vi "Set Scale.vi"(9 "Scale Visible":bool[](array[boolean]), 10 "X坐标轴":T1, 11 "Data Viewer in":refnum<class "Data Viewer.lvclass">) -> (3 "Data Viewer Out":refnum<class "Data Viewer.lvclass">)   [LabVIEW 2020, in "Data Viewer.lvlib" / "Data Viewer.lvclass"]
uses:
  Data Viewer.lvclass
  Data Viewer.lvclass/Data Viewer.ctl
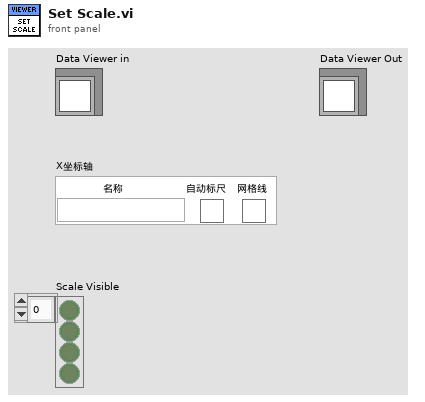
[diagram p1: front panel]
types:
  T1 = cluster{"名称":string, "Auto Scale":bool, "Gird Line":bool}
  T2 = typedef "Data Viewer.lvlib/Data Viewer.lvclass/Scale Setting--cluster.ctl" = cluster{"Name":string, "Unit":string, "Color":u32, "Auto Scale":bool, "Scale Min":dbl, "Scale Max":dbl, "Scale Interval":dbl, "Show Gird":bool, "Log":bool}
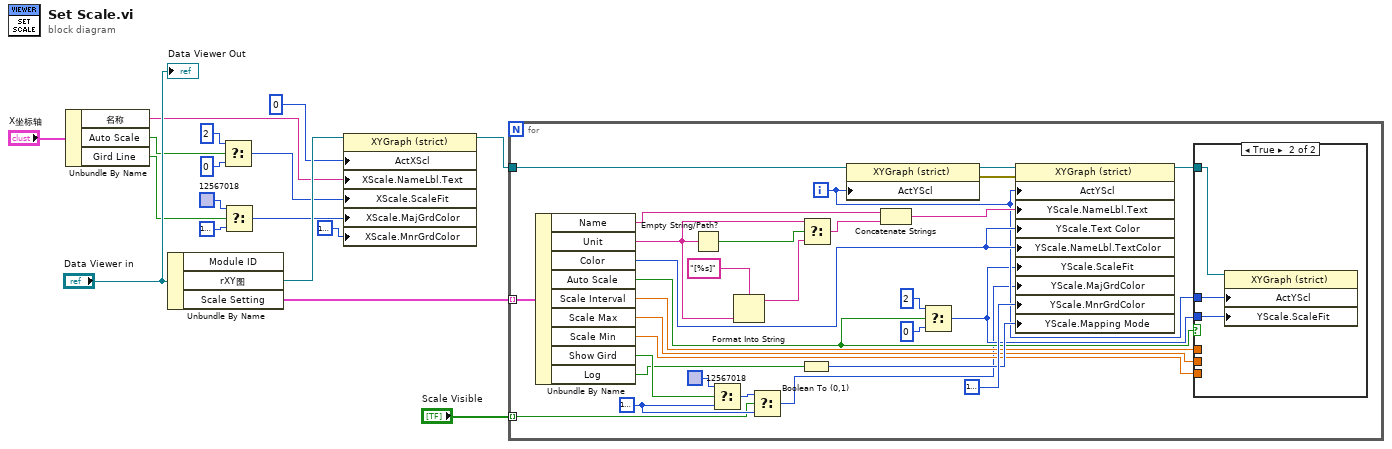
[diagram p0: block diagram]
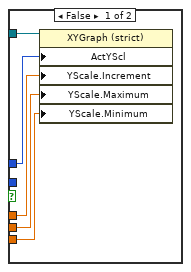
[diagram p2: hidden frame]
diagram:
  n1 = Unbundle By Name("X坐标轴") -> ("名称"=w12:string, "Auto Scale"=w11:bool, "Gird Line"=w6:bool)
  n2 = Unbundle By Name("Data Viewer in") -> ("rXY图"=w15:refnum<vi>, "Scale Setting"=w17:T2[])  [unwired: 1 out]
  n3 = Select(t=u8 2, s=w11, f=u8 0 ("Y Scale.Scale Fit")) -> (s? t:f=w8:u8)
  n4 = Select(t=u32 12567018 ("Y Scale.Grid Colors:Minor Color"), s=w6, f=u32 16777216 ("Y Scale.Grid Colors:Minor Color")) -> (s? t:f=w4:u32)
  n5 = property class="XYGraph (strict)"(reference=w15, "ActXScl"=0 ("Active X Scale"), "XScale.NameLbl.Text"=w12, "XScale.ScaleFit"=w8, "XScale.MajGrdColor"=w4, "XScale.MnrGrdColor"=u32 16777216 ("Y Scale.Grid Colors:Minor Color")) -> (reference out=w2:refnum<vi>)  [unwired: 1 in, 1 out]
  n6 = for {
    tunnel: w17 -> [w47] mode=indexing
    tunnel: w2 -> [w33]
    tunnel: "Scale Visible" -> [w18] mode=indexing
    i -> [w28]
    w20 = u32 16777216 ("Y Scale.Grid Colors:Minor Color")
    n7 = Unbundle By Name(w47) -> ("Name"=w41:string, "Unit"=w44:string, "Color"=w30:u32, "Auto Scale"=w27:bool, "Scale Interval"=w26:dbl, "Scale Max"=w25:dbl, "Scale Min"=w24:dbl, "Show Gird"=w37:bool, "Log"=w36:bool)
    n8 = Empty String/Path?(string/path=w44) -> (empty?=w46:bool)
    n9 = Select(t=u32 12567018 ("Y Scale.Grid Colors:Minor Color"), s=w37, f=w20) -> (s? t:f=w21:u32)
    n10 = Format Into String(format string="[%s]", w44) -> (resulting string=w45:string)  [unwired: 2 in, 1 out]
    n11 = Select(t=w21, s=w18, f=w20) -> (s? t:f=w19:u32)
    n12 = Boolean To (0,1)(Boolean=w36) -> (0, 1=w35:i16)
    n13 = Select(t=w44, s=w46, f=w45) -> (s? t:f=w42:string)
    n14 = property class="XYGraph (strict)"(reference=w33, "ActYScl"=w28) -> (reference out=w31:refnum<vi>, error out=w32:errorcluster)  [unwired: 1 in]
    n15 = Concatenate Strings(w41, w42) -> (w34:string)
    n16 = Select(t=u8 2, s=w27, f=u8 0 ("Y Scale.Scale Fit")) -> (s? t:f=w23:u8)
    n17 = property class="XYGraph (strict)"(reference=w31, error in=w32, "ActYScl"=w28, "YScale.NameLbl.Text"=w34, "YScale.Text Color"=w30, "YScale.NameLbl.TextColor"=w30, "YScale.ScaleFit"=w23, "YScale.MajGrdColor"=w19, "YScale.MnrGrdColor"=u32 16777216 ("Y Scale.Grid Colors:Minor Color"), "YScale.Mapping Mode"=w35) -> (reference out=w29:refnum<vi>)  [unwired: 1 out]
    n18 = case shown="True" w27 {
      tunnel: w29 -> [w52 w55]
      tunnel: w28 -> [w51 w54]
      tunnel: w26 -> [w50 _]
      tunnel: w25 -> [w49 _]
      tunnel: w24 -> [w48 _]
      tunnel: w23 -> [_ w53]
      frame False {
        n19 = property class="XYGraph (strict)"(reference=w52, "ActYScl"=w51, "YScale.Increment"=w50, "YScale.Maximum"=w49, "YScale.Minimum"=w48) -> ()  [unwired: 1 in, 2 out]
      }
      frame True {
        n20 = property class="XYGraph (strict)"(reference=w55, "ActYScl"=w54, "YScale.ScaleFit"=w53) -> ()  [unwired: 1 in, 2 out]
      }
    }
  }
  "Data Viewer Out" <- "Data Viewer in"
